vi "Test My Cloneable Module API.vi"() -> ()   [LabVIEW 2026]
doc: "My Module API Tester.\n_____\nBased on DQMH Dev Tools: Project Template 7.1.2.1547."
uses:
  My Cloneable Module.lvlib
  <vilib>/Utility/error.llb/DialogType.ctl
  <vilib>/Utility/error.llb/Search and Replace Pattern (string).vi
panel:
  in  "String":string
  in  "Request a HL":bool
  out "Map":map{i32, string}(c390)
  in  "IP":string
  out "last error":errorcluster
  in  "Show Diagram on Init":bool
  in  "wait for reply":bool=TRUE
  in  "Run as Singleton?":bool
  in  "Show Block Diagram":bool
  in  "Refresh Modules":bool
  in  "X":dbl=1.0
  out "Reply Payload":dbl
  out "Active Modules":string[](array[string])
  in  "Stop Module":bool
  in  "Select Module":i32(ring)=-1 caption="Select Module\nTo send Request to" items=["All"=-1, "2"=2, "3"=3]
  in  "Run New Module":bool
  out "Do Something Count":i32
  in  "Test Do Something Else and Wait for Reply":bool
  in  "Hide Module Panel":bool
  in  "Show Module Panel":bool
  in  "Test Do Something Else":bool
  in  "Test Do Something":bool
  out "Status":string
  # "This VI tests the API for the Module."
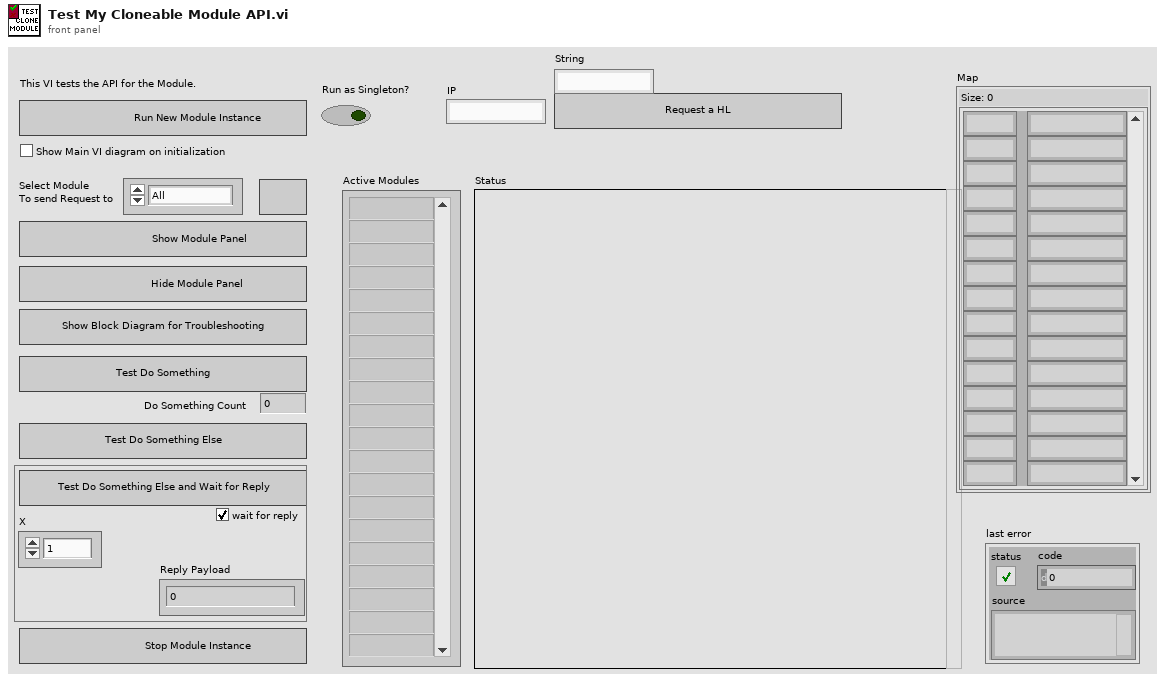
[diagram p1: front panel]
types:
  T1 = typedef "My Cloneable Module.lvlib/Broadcast Events--cluster.ctl" = cluster{"Module Did Init":refnum<user-event>, "Status Updated":refnum<user-event>, "Error Reported":refnum<user-event>, "Did Something":refnum<user-event>, "Module Did Stop":refnum<user-event>, "Update Module Execution Status":refnum<user-event>}
  T2 = typedef "DialogType.ctl" = u16
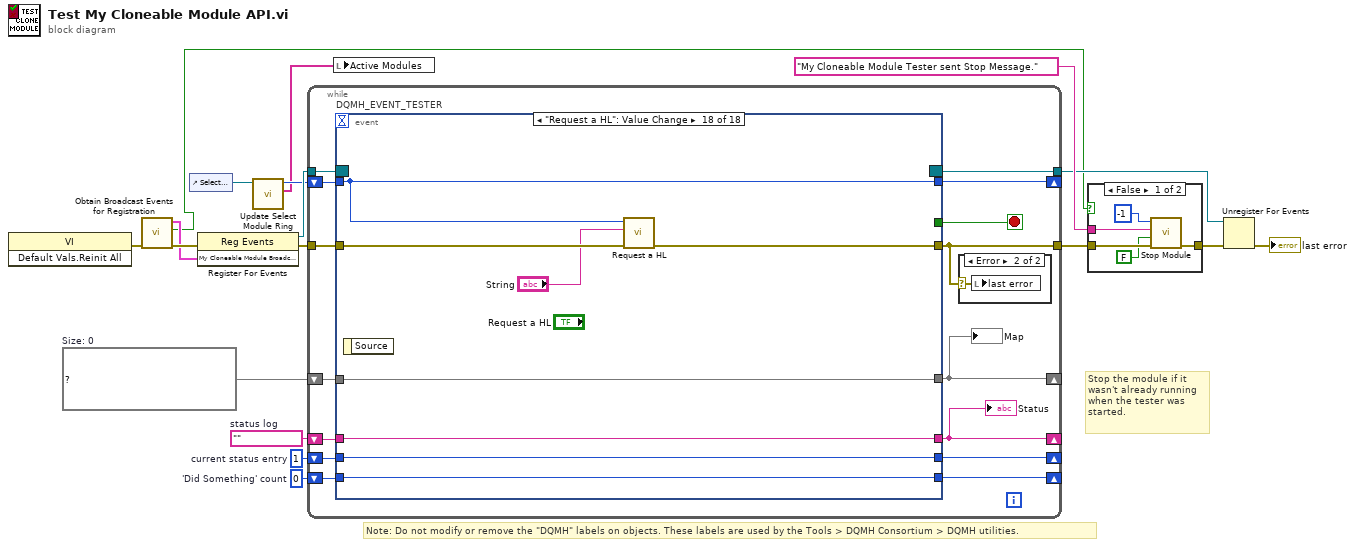
[diagram p0: block diagram]
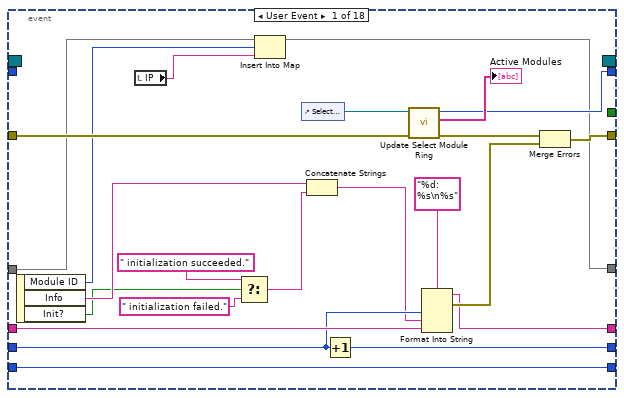
[diagram p4: hidden frame]
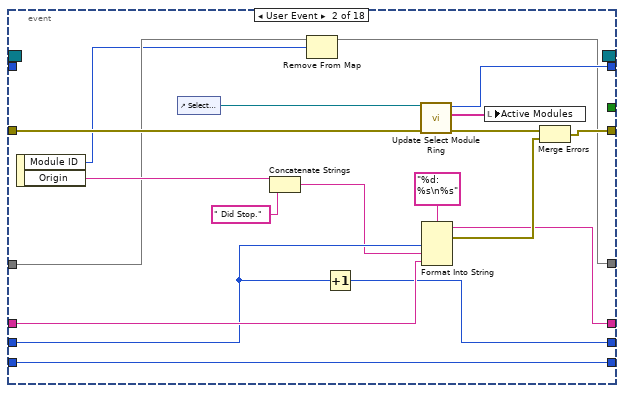
[diagram p5: hidden frame]
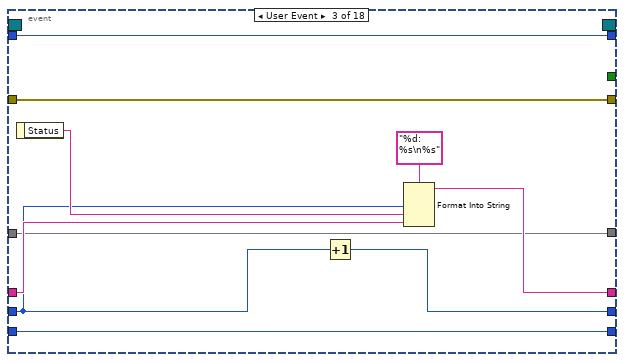
[diagram p6: hidden frame]
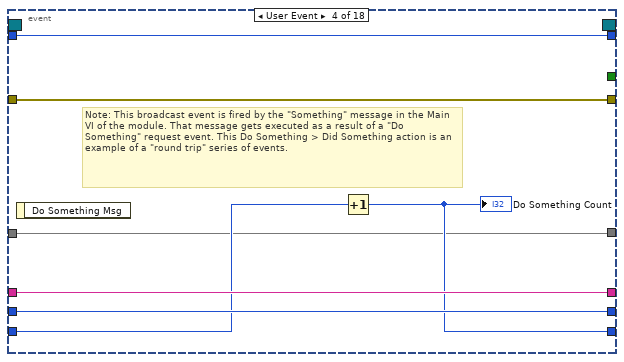
[diagram p7: hidden frame]
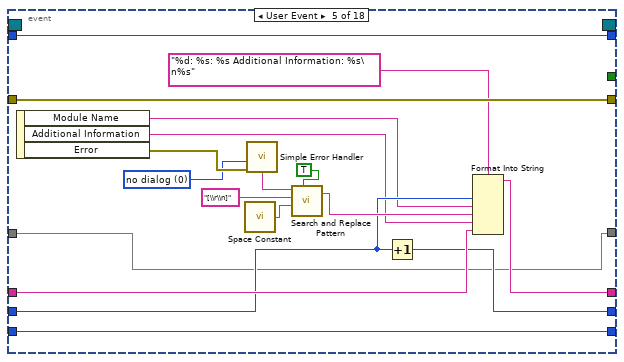
[diagram p8: hidden frame]
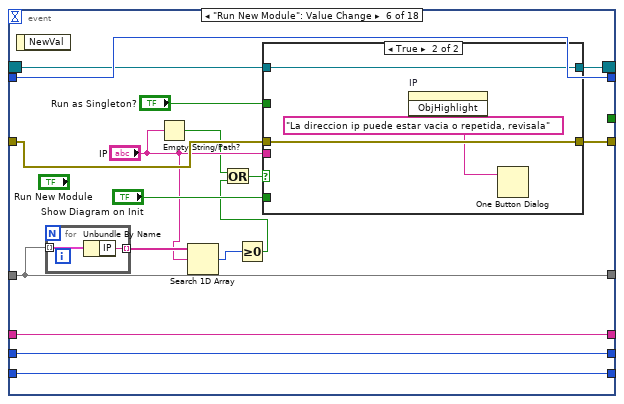
[diagram p9: hidden frame]
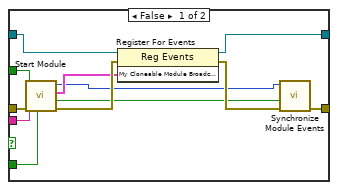
[diagram p10: hidden frame]
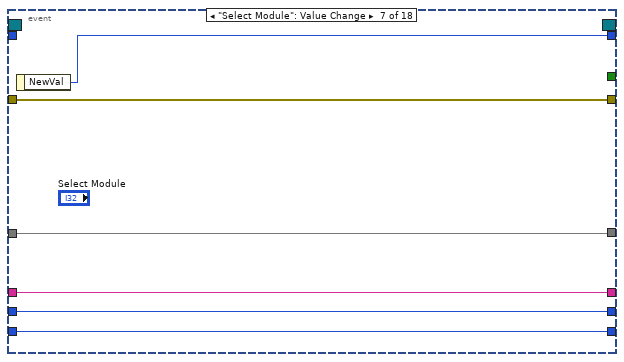
[diagram p11: hidden frame]
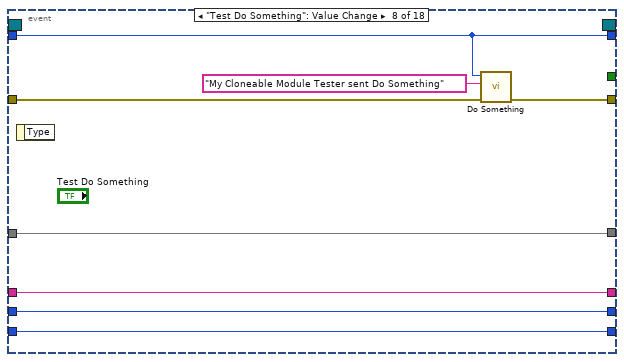
[diagram p12: hidden frame]
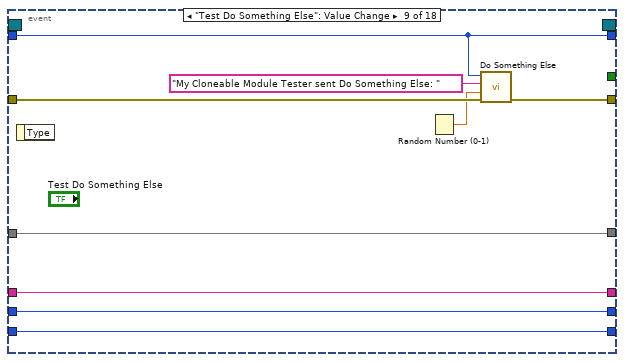
[diagram p13: hidden frame]
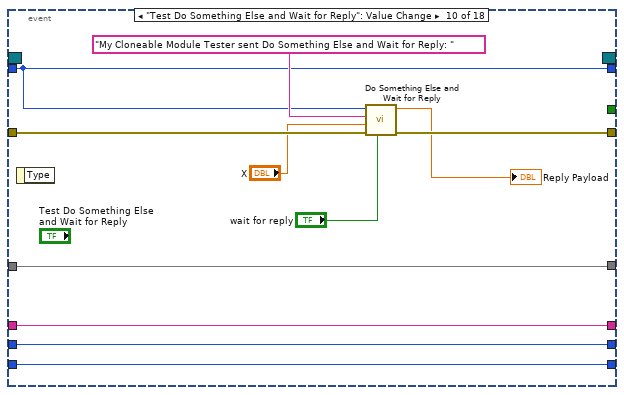
[diagram p14: hidden frame]
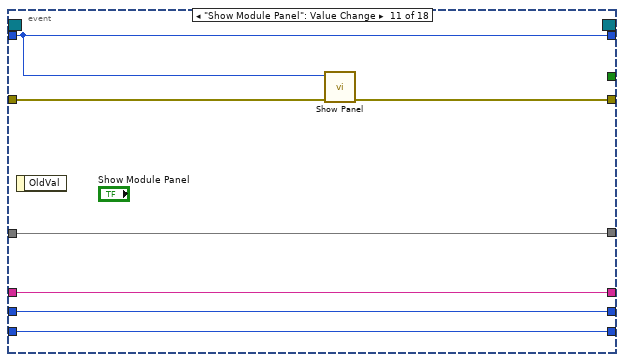
[diagram p15: hidden frame]
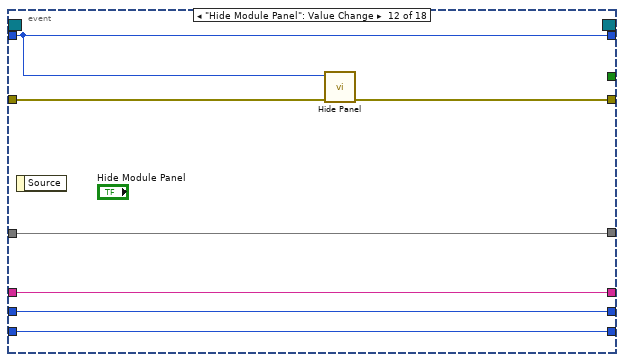
[diagram p16: hidden frame]
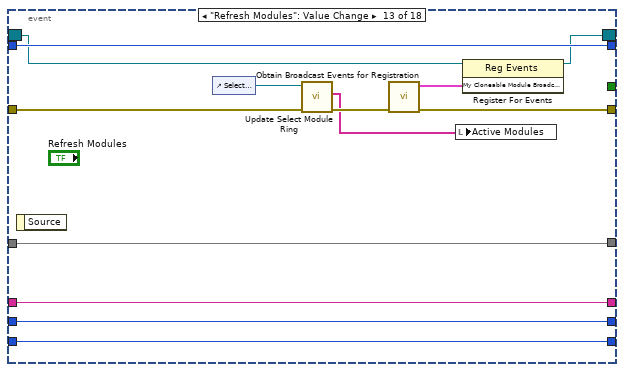
[diagram p17: hidden frame]
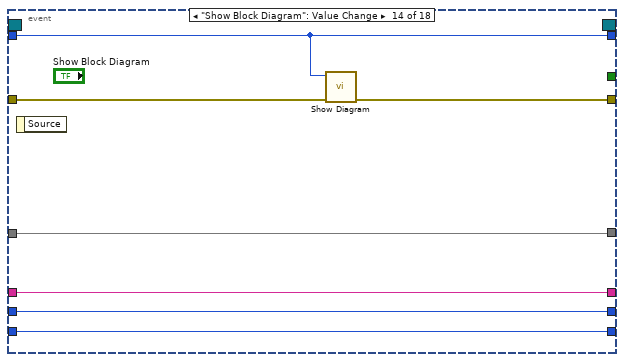
[diagram p18: hidden frame]
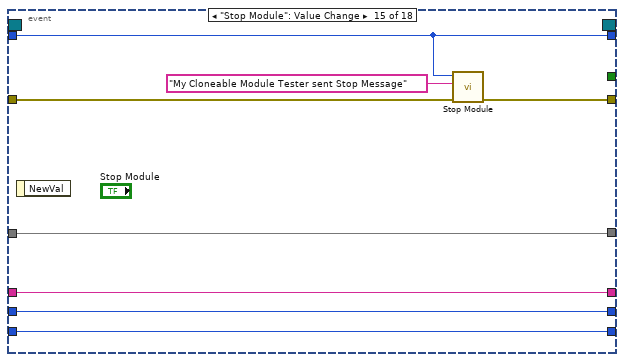
[diagram p19: hidden frame]
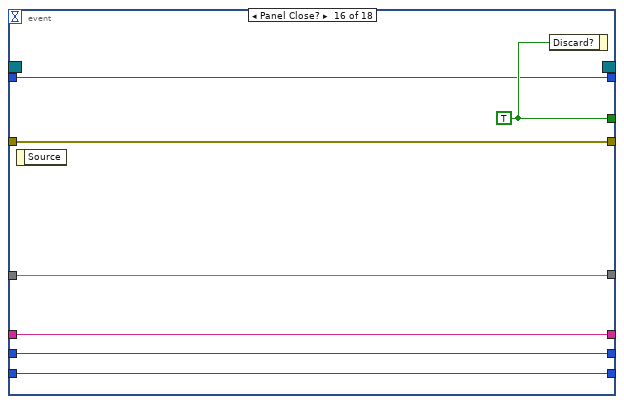
[diagram p20: hidden frame]
diagram:
  w1 = map{i32, string} {}  # Size: 0
  w9 = 0  # 'Did Something' count
  w10 = 1  # current status entry
  w11 = ""  # status log
  # "Stop the module if it wasn't already running when the tester was started."
  # "Note: Do not modify or remove the \"DQMH\" labels on objects. These labels are used by the Tools > DQMH Consortium > DQMH utilities."
  n1 = invoke on="Invoke Node" class="VI" method="Default Vals.Reinit All"() -> (error out=w16:errorcluster)  [unwired: 3 in, 2 out]
  n2 = call "Obtain Broadcast Events for Registration.vi"("error in"=w16) -> ("error out"=w15:errorcluster, "Already running?"=w5:bool, "My Cloneable Module Broadcast Events"=w8:T1)  [unwired: 8 in]
  n3 = control-ref of="Select Module"() -> (w4:refnum<vi>)
  n4 = register-events(error in=w15, w8) -> (reference out=w12:refnum<event-registration>, error out=w17:errorcluster)  [unwired: 1 in]
  n5 = call "Update Select Module Ring.vi"("Select Module Ring Ref"=w4) -> ("Active Modules (Array)"=w2:string[], "New Module Ring Value"=w3:i32)  [unwired: 8 in, 1 out]
  n6 = while {
    tunnel: w12 -> [w31]
    tunnel: [w32] -> w14
    tunnel: w17 -> [w33]
    shift-right: [w27] -> _
    shift-left: w11 -> [w29]
    shift-right: [w28] -> _
    shift-left: w10 -> [w30]
    shift-right: [w25] -> _
    shift-left: w9 -> [w26]
    shift-right: [w23] -> _
    shift-left: w3 -> [w24]
    tunnel: [w22] -> w6
    shift-right: [w19] -> _
    shift-left: w1 -> [w20]
    stop <- w21 stop-if-true
    n7 = event "DQMH_EVENT_TESTER" shown="[17] \"Request a HL\": Value Change" {
      selector: w31 -> [_ _ _ _ _ w122 _ _ _ _ _ _ w198 _ _ _ _ _]
      dyn-events: [_ _ _ _ _ w121 _ _ _ _ _ _ w197 _ _ _ _ _] -> w22
      timeout: _ -> [_ _ _ _ _ _ _ _ _ _ _ _ _ _ _ _ _ _]
      tunnel: [_ _ _ _ _ _ _ _ _ _ _ _ _ _ _ w227 _ _] -> w21
      tunnel: [w54 w73 w86 w93 w111 w127 w151 w158 w167 w179 w185 w192 w204 w212 w220 w228 w236 w239] -> w32
      tunnel: w33 -> [w56 w75 w86 w93 w111 w128 w151 w159 w168 w178 w186 w193 w206 w213 w221 w228 w237 w245]
      tunnel: w30 -> [w51 w70 w78 w91 w99 w125 w149 w155 w163 w175 w183 w190 w202 w210 w218 w225 w234 w243]
      tunnel: w29 -> [w52 w71 w82 w92 w100 w126 w150 w156 w164 w176 w184 w191 w203 w211 w219 w226 w235 w244]
      tunnel: [w49 w68 w83 w92 w98 w126 w150 w156 w164 w176 w184 w191 w203 w211 w219 w226 w235 w244] -> w27
      tunnel: [w50 w69 w85 w91 w97 w125 w149 w155 w163 w175 w183 w190 w202 w210 w218 w225 w234 w243] -> w28
      tunnel: w26 -> [w46 w67 w81 w90 w109 w124 w148 w154 w162 w174 w182 w189 w201 w209 w217 w224 w233 w242]
      tunnel: [w46 w67 w81 w89 w109 w124 w148 w154 w162 w174 w182 w189 w201 w209 w217 w224 w233 w242] -> w25
      tunnel: w24 -> [_ _ w79 w88 w108 w123 _ w153 w161 w173 w181 w188 w200 w208 w216 w223 _ w241]
      tunnel: [w43 w64 w79 w88 w108 w123 w147 w153 w161 w173 w181 w188 w200 w208 w216 w223 w231 w241] -> w23
      tunnel: w20 -> [w38 w60 w77 w87 w94 w118 w146 w152 w160 w169 w180 w187 w194 w207 w214 w222 w229 w240]
      tunnel: [w37 w58 w77 w87 w94 w118 w146 w152 w160 w169 w180 w187 w194 w207 w214 w222 w229 w240] -> w19
      event User Event {
        n8 = event-data() -> ("Module ID"=w36:i32, "Info"=w48:string, "Init?"=w40:bool)  [unwired: 1 in]
        n9 = local read "IP"() -> (w35:string)
        n10 = Select(t=" initialization succeeded.", s=w40, f=" initialization failed.") -> (s? t:f=w39:string)
        n11 = Insert Into Map(map in=w38, key=w36, value=w35) -> (map out=w37:map{i32, string})  [unwired: 2 out]
        n12 = control-ref of="Select Module"() -> (w45:refnum<vi>)
        n13 = Concatenate Strings(w48, w39) -> (w47:string)
        n14 = Increment(x=w51) -> (x+1=w50:i32)
        n15 = call "Update Select Module Ring.vi"("error in"=w56, "Select Module Ring Ref"=w45) -> ("error out"=w55:errorcluster, "Active Modules (Array)"=→"Active Modules":string[], "New Module Ring Value"=w43:i32)  [unwired: 7 in]
        n16 = Format Into String(format string="%d: %s\n%s", w51, w47, w52) -> (resulting string=w49:string, error out=w57:errorcluster)  [unwired: 2 in]
        n17 = Merge Errors(w55, w57) -> (w54:errorcluster)
      }
      event User Event {
        n18 = event-data() -> ("Module ID"=w59:i32, "Origin"=w62:string)  [unwired: 1 in]
        n19 = control-ref of="Select Module"() -> (w66:refnum<vi>)
        n20 = Concatenate Strings(w62, " Did Stop.") -> (w61:string)
        n21 = Remove From Map(10:w59, 11:w60) -> (3:w58:map{i32, string})  [unwired: 2 out]
        n22 = Increment(x=w70) -> (x+1=w69:i32)
        n23 = call "Update Select Module Ring.vi"("error in"=w75, "Select Module Ring Ref"=w66) -> ("error out"=w74:errorcluster, "Active Modules (Array)"=w65:string[], "New Module Ring Value"=w64:i32)  [unwired: 7 in]
        n24 = Format Into String(format string="%d: %s\n%s", w70, w61, w71) -> (resulting string=w68:string, error out=w76:errorcluster)  [unwired: 2 in]
        n25 = local write "Active Modules"(w65) -> ()
        n26 = Merge Errors(w74, w76) -> (w73:errorcluster)
      }
      event User Event {
        n27 = event-data() -> ("Status"=w80:string)  [unwired: 1 in]
        n28 = Increment(x=w78) -> (x+1=w85:i32)
        n29 = Format Into String(format string="%d: %s\n%s", w78, w80, w82) -> (resulting string=w83:string)  [unwired: 2 in, 1 out]
      }
      event User Event {
        # "Note: This broadcast event is fired by the \"Something\" message in the Main VI of the module. That message gets executed as a result of a \"Do Something\" request event. This Do Something > Did Something action is an example of a \"round trip\" series of events."
        n30 = event-data() -> ()  [unwired: 1 in, 1 out]
        n31 = Increment(x=w90) -> (x+1=w89:i32)
        "Do Something Count" <- w89
      }
      event User Event {
        w101 = T2 0 items=["no dialog", "OK message", "continue or stop message", "OK message + warnings", "continue/stop + warnings"] ("type of dialog (OK msg:1)")
        n32 = event-data() -> ("Module Name"=w96:string, "Additional Information"=w95:string, "Error"=w110:errorcluster)  [unwired: 1 in]
        n33 = call <vilib>:"Space Constant.vi"() -> ("String"=w105:string)
        n34 = call <vilib>:"Simple Error Handler.vi"("type of dialog (OK msg:1)"=w101, "error in (no error)"=w110) -> ("message"=w102:string)  [unwired: 3 in, 4 out]
        n35 = call-poly <vilib>:"Search and Replace Pattern.vi"("string"=w102, "regular expression (\"\")"="[\\r\\n]" ("regular expression (\"\")"), "replace string (\"\")"=w105, "replace all? (F)"=TRUE ("replace all CR/LF with spaces")) -> ("result string"=w103:string)  [unwired: 1 in, 1 out]
        n36 = Increment(x=w99) -> (x+1=w97:i32)
        n37 = Format Into String(format string="%d: %s: %s Additional Information: %s\n%s", w99, w96, w103, w95, w100) -> (resulting string=w98:string)  [unwired: 2 in, 1 out]
      }
      event "Run New Module": Value Change {
        n38 = event-data() -> ()  [unwired: 1 in, 1 out]
        n39 = for {
          tunnel: w118 -> [w130] mode=indexing
          tunnel: [w129] -> w117 mode=indexing
          n40 = Unbundle By Name(w130) -> ("IP"=w129:string)
        }
        n41 = Empty String/Path?(string/path="IP") -> (empty?=w114:bool)
        n42 = Search 1D Array(1D array=w117, element="IP") -> (index of element=w115:i32)  [unwired: 1 in]
        n43 = Greater Or Equal To 0?(x=w115) -> (x >= 0?=w113:bool)
        n44 = Or(x=w114, y=w113) -> (x .or. y?=w112:bool)
        n45 = case shown="True" w112 {
          tunnel: w128 -> [w140 w145]
          tunnel: w122 -> [w138 w144]
          tunnel: [w137 w144] -> w121
          tunnel: [w139 w145] -> w127
          tunnel: "Run as Singleton?" -> [w134 _]
          tunnel: "Show Diagram on Init" -> [w133 _]
          tunnel: "IP" -> [w131 _]
          frame False {
            n46 = call "Start Module.vi"("Show Main VI Diagram on Init (F)"=w133, "error in"=w140, "IP"=w131, "Run as Singleton? (F)"=w134) -> ("error out"=w141:errorcluster, "Wait for Event Sync?"=w136:bool, "My Cloneable Module Broadcast Events"=w135:T1, "Module ID"=w132:i32)  [unwired: 3 in, 1 out]
            n47 = register-events(reference=w138, error in=w141, w135) -> (reference out=w137:refnum<event-registration>, error out=w142:errorcluster)
            n48 = call "Synchronize Module Events.vi"("error in"=w142, "Wait for Event Sync?"=w136, "Module ID in"=w132) -> ("error out"=w139:errorcluster)  [unwired: 7 in, 1 out]
          }
          frame True {
            n49 = invoke on="IP" class="Str" method="ObjHighlight"() -> ()  [unwired: 3 in, 3 out]
            n50 = One Button Dialog(message="La direccion ip puede estar vacia o repetida, revisala") -> ()  [unwired: 1 in, 1 out]
          }
        }
      }
      event "Select Module": Value Change {
        n51 = event-data() -> ("NewVal"=w147:i32)  [unwired: 1 in]
      }
      event "Test Do Something": Value Change {
        n52 = event-data() -> ()  [unwired: 1 in, 1 out]
        n53 = call "Do Something.vi"("error in"=w159, "Do Something Message"="My Cloneable Module Tester sent Do Something", "Module ID"=w153) -> ("error out"=w158:errorcluster)  [unwired: 8 in]
      }
      event "Test Do Something Else": Value Change {
        n54 = event-data() -> ()  [unwired: 1 in, 1 out]
        n55 = Random Number (0-1)() -> (number: 0 to 1=w165:dbl)
        n56 = call "Do Something Else.vi"("error in"=w168, "X"=w165, "Do Something else Message"="My Cloneable Module Tester sent Do Something Else: " ("Do Something Message"), "Module ID"=w161) -> ("error out"=w167:errorcluster)  [unwired: 7 in]
      }
      event "Test Do Something Else and Wait for Reply": Value Change {
        n57 = event-data() -> ()  [unwired: 1 in, 1 out]
        n58 = call "Do Something Else and Wait for Reply.vi"("wait for reply (T)"="wait for reply", "error in"=w178, "X"="X", "Do Something Else Message"="My Cloneable Module Tester sent Do Something Else and Wait for Reply: " ("Do Something Message"), "Module ID"=w173) -> ("error out"=w179:errorcluster, "Value"=→"Reply Payload":dbl)  [unwired: 4 in, 1 out]
      }
      event "Show Module Panel": Value Change {
        n59 = event-data() -> ()  [unwired: 1 in, 1 out]
        n60 = call "Show Panel.vi"("error in"=w186, "Module ID"=w181) -> ("error out"=w185:errorcluster)  [unwired: 9 in]
      }
      event "Hide Module Panel": Value Change {
        n61 = event-data() -> ()  [unwired: 1 in, 1 out]
        n62 = call "Hide Panel.vi"("error in"=w193, "Module ID"=w188) -> ("error out"=w192:errorcluster)  [unwired: 9 in]
      }
      event "Refresh Modules": Value Change {
        n63 = event-data() -> ()  [unwired: 1 in, 1 out]
        n64 = control-ref of="Select Module"() -> (w199:refnum<vi>)
        n65 = call "Update Select Module Ring.vi"("error in"=w206, "Select Module Ring Ref"=w199) -> ("error out"=w205:errorcluster, "Active Modules (Array)"=w195:string[])  [unwired: 7 in, 1 out]
        n66 = call "Obtain Broadcast Events for Registration.vi"("error in"=w205) -> ("error out"=w204:errorcluster, "My Cloneable Module Broadcast Events"=w196:T1)  [unwired: 8 in, 1 out]
        n67 = local write "Active Modules"(w195) -> ()
        n68 = register-events(reference=w198, w196) -> (reference out=w197:refnum<event-registration>)  [unwired: 1 in, 1 out]
      }
      event "Show Block Diagram": Value Change {
        n69 = event-data() -> ()  [unwired: 1 in, 1 out]
        n70 = call "Show Diagram.vi"("error in"=w213, "Module ID"=w208) -> ("error out"=w212:errorcluster)  [unwired: 9 in]
      }
      event "Stop Module": Value Change {
        n71 = event-data() -> ()  [unwired: 1 in, 1 out]
        n72 = call "Stop Module.vi"("error in"=w221, "Origin"="My Cloneable Module Tester sent Stop Message", "Module ID"=w216) -> ("error out"=w220:errorcluster)  [unwired: 8 in]
      }
      event Panel Close? {
        w227 = TRUE ("Discard?")
        n73 = event-data() -> ()  [unwired: 1 in, 1 out]
        n74 = event-data ("Event Filter Node")("Discard?"=w227) -> ()  [unwired: 1 in, 1 out]
      }
      event User Event {
        # "Update the active modules list whenever the module execution status is updated. Note that this event should only ever fire when Start Module VI is called for a cloneable running as singleton, but the module is already running."
        n75 = event-data() -> ()  [unwired: 1 in, 1 out]
        n76 = control-ref of="Select Module"() -> (w232:refnum<vi>)
        n77 = call "Update Select Module Ring.vi"("error in"=w237, "Select Module Ring Ref"=w232) -> ("error out"=w236:errorcluster, "Active Modules (Array)"=w230:string[], "New Module Ring Value"=w231:i32)  [unwired: 7 in]
        n78 = local write "Active Modules"(w230) -> ()
      }
      event "Request a HL": Value Change {
        n79 = event-data() -> ()  [unwired: 1 in, 1 out]
        n80 = call "Request a HL.vi"("error in"=w245, "String"="String", "Module ID"=w241) -> ("error out"=w239:errorcluster)  [unwired: 8 in]
      }
    }
    "Status" <- w27
    "Map" <- w19
    n81 = case shown="Error" w32 {
      selector: w32 -> [_ w34]
      frame No Error {
      }
      frame Error {
        n82 = local write "last error"(w34) -> ()
      }
    }
  }
  n83 = local write "Active Modules"(w2) -> ()
  n84 = case shown="False" w5 {
    tunnel: [w250 w251] -> w18
    tunnel: "My Cloneable Module Tester sent Stop Message." ("Origin") -> [w248 _]
    tunnel: w14 -> [w249 w251]
    frame False {
      n85 = call "Stop Module.vi"("error in"=w249, "Wait for Module to stop? (F)"=FALSE ("Wait for Module to stop?"), "Origin"=w248, "Module ID"=-1 ("Stop all")) -> ("error out"=w250:errorcluster)  [unwired: 7 in]
    }
    frame True {
    }
  }
  n86 = Unregister For Events(event registration refnum=w6, error in=w18) -> (error out=→"last error":errorcluster)
